vi "Test - Check.vi"(8 "error in (no error)":errorcluster, 9 "Condition":bool, 10 "Check Name":string, 11 "Report in":string) -> (0 "error out":errorcluster, 3 "Report out":string)   [LabVIEW 2024]
doc: "Appends one line \"PASS: <Check Name>\" or \"FAIL: <Check Name>\" to Report, depending on Condition.\n\nGenerated by: Claude"
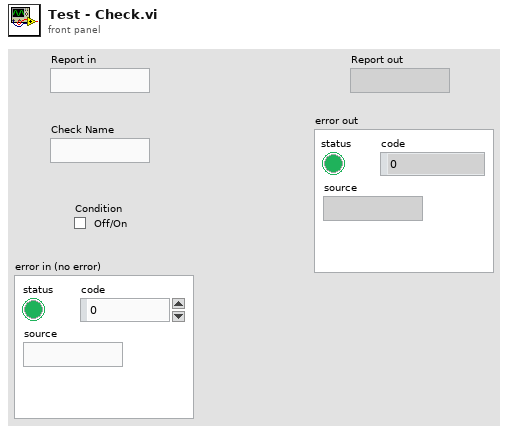
[diagram p1: front panel]
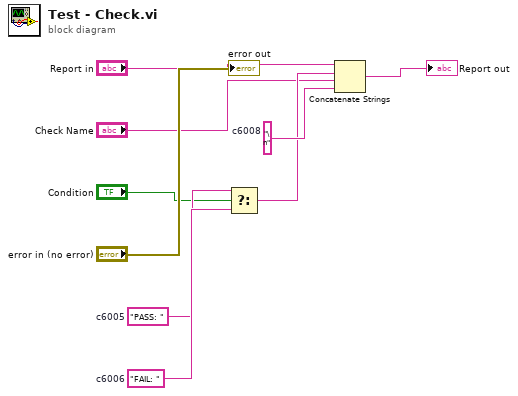
[diagram p0: block diagram]
diagram:
  w8 = "\n"  # c6008
  w6 = "FAIL: "  # c6006
  w5 = "PASS: "  # c6005
  n1 = Select(t=w5, s="Condition", f=w6) -> (s? t:f=w7:string)
  n2 = Concatenate Strings("Report in", w7, "Check Name", w8) -> (→"Report out":string)
  "error out" <- "error in (no error)"
